vi "Database-ref.vi"(7 "枚举":enum16{"W", "R"}(ring)=enum."R", 11 "connection reference":T1) -> (3 "connection reference out":T1)   [LabVIEW 2025, in "Database_access.lvclass"]
uses:
  Database_access.lvclass
  <vilib>/addons/database/Connection.llb/Conn ObjectReference.ctl
  <vilib>/addons/database/NI_Database_API.lvlib
panel:
  # "仅为方便程序使用，\n请不要使用这个FGV"
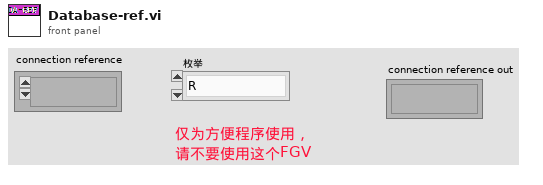
[diagram p1: front panel]
types:
  T1 = typedef "NI_Database_API.lvlib/Conn ObjectReference.ctl" = refnum<k1>
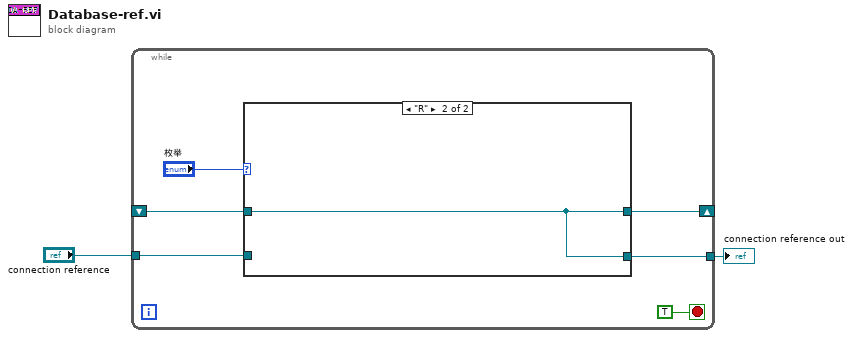
[diagram p0: block diagram]
diagram:
  n1 = while {
    shift-right: [w5] -> _
    shift-left: _ -> [w3]
    tunnel: "connection reference" -> [w6]
    tunnel: [w4] -> w1
    stop <- TRUE stop-if-true
    n2 = case shown="\"R\"" "枚举" {
      tunnel: w6 -> [w9 _]
      tunnel: [w9 w10] -> w5
      tunnel: [w9 w10] -> w4
      tunnel: w3 -> [_ w10]
      frame "W", Default {
      }
      frame "R" {
      }
    }
  }
  "connection reference out" <- w1
